vi "test server discover.vi"(8 "error in (no error)":errorcluster) -> (0 "error out":errorcluster, 3 "body":string)   [LabVIEW 2020, in "MCP Server tests.lvlib"]
doc: "server/discover (modern only) answers resultType complete, supportedVersions (all versions: 2026-07-28 and the legacy ones including 2025-11-25), the capabilities that initialize reports, _meta serverInfo and the caching hints. initialize stays legacy: asked for 2026-07-28 it answers the newest legacy version 2025-11-25, and 2025-11-25 is negotiable. The requests are sent with the LabVIEW HTTP Client directly."
uses:
  MCP Server tests.lvlib
  671d1c08-5dc6-4caa-967e-c1c9fcee9c7e.vi
  <vilib>/JDP Science/JSONtext/Next JSON Value.vi
  <vilib>/JDP Science/JSONtext/String Subset.vi
  <vilib>/JDP Science/JSONtext/Parsing/Advance past next JSON Value (inlined COPY).vi
  <vilib>/JDP Science/JSONtext/Parsing/Advance past whitespace.vi
  <vilib>/JDP Science/JSONtext/Parsing/Advance past String.vi
  <vilib>/JDP Science/JSONtext/Parsing/Advance past Number.vi
  <vilib>/JDP Science/JSONtext/Parsing/Advance past Line Ending.vi
  <vilib>/JDP Science/JSONtext/Parsing/Parse Full Path or Item Name.vi
  <vilib>/JDP Science/JSONtext/Parsing/Advance past Array.vi
  <vilib>/JDP Science/JSONtext/Parsing/Advance past Object.vi
  <vilib>/JDP Science/JSONtext/support/Error Cluster From Code.vi
  <vilib>/JDP Science/JSONtext/Offset/Find Item Locations by Path.vi
  <vilib>/JDP Science/JSONtext/JSON text to Variant.vi
  <vilib>/JDP Science/JSONtext/LVClass Serializer/JSONtext LVClass Serializer.lvclass
  <vilib>/addons/_JKI Toolkits/Caraya/classes/Test/Test.lvclass
  <vilib>/JDP Science/JSONtext/JSONtext.lvlib
  <vilib>/addons/_JKI Toolkits/Caraya/classes/Assert/Assert.lvclass
panel:
  out "lookup error":errorcluster
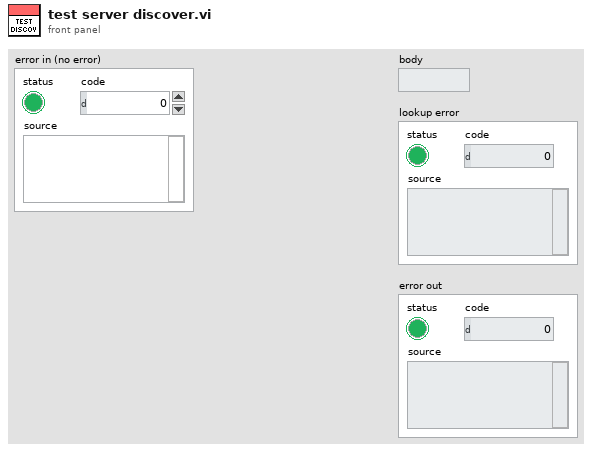
[diagram p1: front panel]
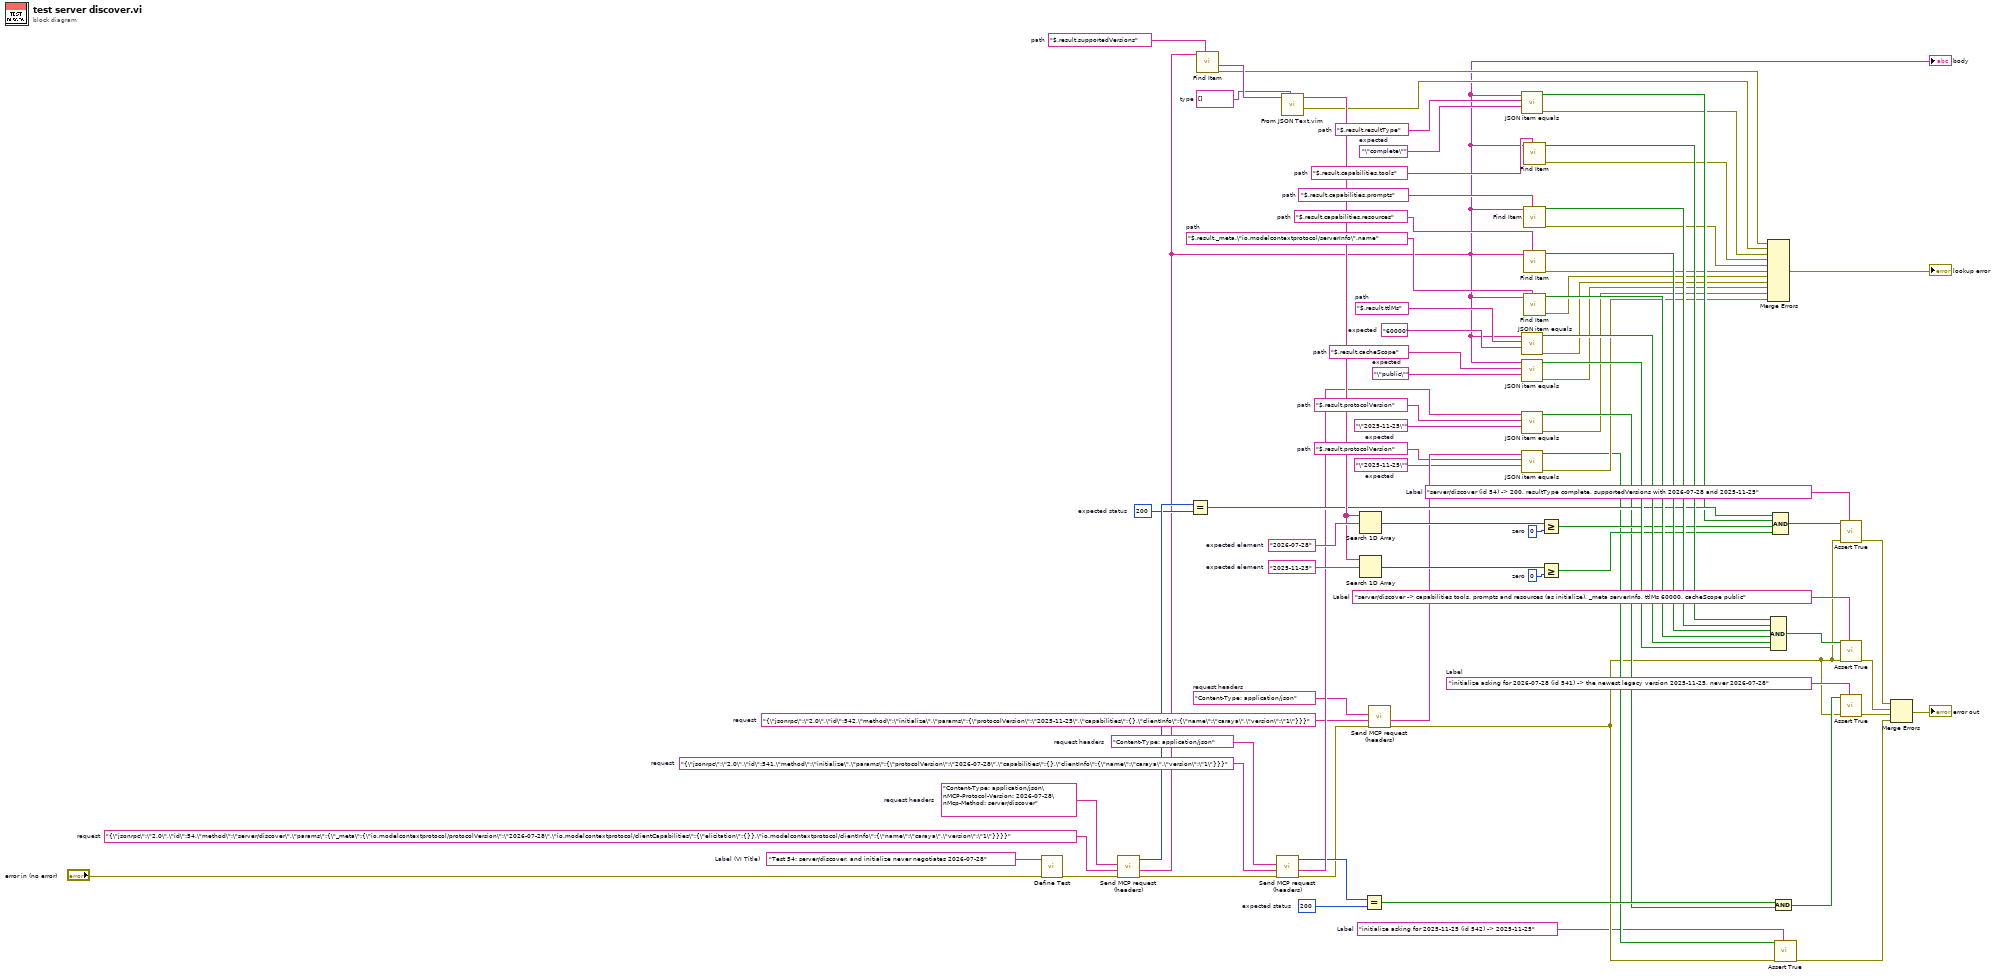
[diagram p0: block diagram]
diagram:
  w33 = "Content-Type: application/json"  # request headers
  w47 = "Content-Type: application/json"  # request headers
  w78 = "Content-Type: application/json\nMCP-Protocol-Version: 2026-07-28\nMcp-Method: server/discover"  # request headers
  w8 = "initialize asking for 2025-11-25 (id 542) -> 2025-11-25"  # Label
  w11 = "initialize asking for 2026-07-28 (id 541) -> the newest legacy version 2025-11-25, never 2026-07-28"  # Label
  w13 = "server/discover -> capabilities tools, prompts and resources (as initialize), _meta serverInfo, ttlMs 60000, cacheScope public"  # Label
  w15 = "server/discover (id 54) -> 200, resultType complete, supportedVersions with 2026-07-28 and 2025-11-25"  # Label
  w18 = "\"2025-11-25\""  # expected
  w19 = "$.result.protocolVersion"  # path
  w38 = "\"2025-11-25\""  # expected
  w39 = "$.result.protocolVersion"  # path
  w36 = 200  # expected status
  w63 = "\"public\""  # expected
  w64 = "$.result.cacheScope"  # path
  w65 = "60000"  # expected
  w66 = "$.result.ttlMs"  # path
  w71 = "$.result._meta.\"io.modelcontextprotocol/serverInfo\".name"  # path
  w72 = "$.result.capabilities.resources"  # path
  w73 = "$.result.capabilities.prompts"  # path
  w74 = "$.result.capabilities.tools"  # path
  w67 = "\"complete\""  # expected
  w68 = "$.result.resultType"  # path
  w61 = 200  # expected status
  w48 = 0  # zero
  w58 = "2025-11-25"  # expected element
  w50 = 0  # zero
  w60 = "2026-07-28"  # expected element
  w69 = string[] []  # type
  w75 = "$.result.supportedVersions"  # path
  w32 = "{\"jsonrpc\":\"2.0\",\"id\":542,\"method\":\"initialize\",\"params\":{\"protocolVersion\":\"2025-11-25\",\"capabilities\":{},\"clientInfo\":{\"name\":\"caraya\",\"version\":\"1\"}}}"  # request
  w46 = "{\"jsonrpc\":\"2.0\",\"id\":541,\"method\":\"initialize\",\"params\":{\"protocolVersion\":\"2026-07-28\",\"capabilities\":{},\"clientInfo\":{\"name\":\"caraya\",\"version\":\"1\"}}}"  # request
  w77 = "{\"jsonrpc\":\"2.0\",\"id\":54,\"method\":\"server/discover\",\"params\":{\"_meta\":{\"io.modelcontextprotocol/protocolVersion\":\"2026-07-28\",\"io.modelcontextprotocol/clientCapabilities\":{\"elicitation\":{}},\"io.modelcontextprotocol/clientInfo\":{\"name\":\"caraya\",\"version\":\"1\"}}}}"  # request
  w80 = "Test 54: server/discover, and initialize never negotiates 2026-07-28"  # Label (VI Title)
  n1 = call <vilib>:"Define Test.vi"("error in (no error)"="error in (no error)", "Label (VI Title)"=w80) -> ("error out"=w76:errorcluster)  [unwired: 8 in, 1 out]
  n2 = call "Send MCP request (headers).vi"("error in (no error)"=w76, "request"=w77, "request headers"=w78) -> ("error out"=w45:errorcluster, "response"=w3:string, "status code"=w62:i32)  [unwired: 5 in, 1 out]
  "body" <- w3
  n3 = Equal?(x=w62, y=w61) -> (x = y?=w44:bool)
  n4 = call <vilib>:"Find Item.vi"("$Path or Item Name"=w75, "JSON"=w3) -> ("error out"=w30:errorcluster, "<JSON>"=w70:string)  [unwired: 6 in, 2 out]
  n5 = call "Send MCP request (headers).vi"("error in (no error)"=w45, "request"=w46, "request headers"=w47) -> ("error out"=w31:errorcluster, "response"=w40:string, "status code"=w37:i32)  [unwired: 5 in, 1 out]
  n6 = call "From JSON Text.vim"("Data Type and Default Value"=w69, "JSON"=w70) -> ("error out"=w29:errorcluster, "Data out"=w59:string[])  [unwired: 8 in]
  n7 = Search 1D Array(1D array=w59, element=w60) -> (index of element=w51:i32)  [unwired: 1 in]
  n8 = Search 1D Array(1D array=w59, element=w58) -> (index of element=w49:i32)  [unwired: 1 in]
  n9 = Equal?(x=w37, y=w36) -> (x = y?=w35:bool)
  n10 = call "Send MCP request (headers).vi"("error in (no error)"=w31, "request"=w32, "request headers"=w33) -> ("error out"=w9:errorcluster, "response"=w20:string)  [unwired: 5 in, 2 out]
  n11 = call "JSON item equals.vi"("expected"=w67, "path"=w68, "JSON"=w3) -> ("error out"=w28:errorcluster, "equal?"=w43:bool)  [unwired: 6 in, 1 out]
  n12 = call "JSON item equals.vi"("expected"=w65, "path"=w66, "JSON"=w3) -> ("error out"=w23:errorcluster, "equal?"=w53:bool)  [unwired: 6 in, 1 out]
  n13 = call "JSON item equals.vi"("expected"=w63, "path"=w64, "JSON"=w3) -> ("error out"=w22:errorcluster, "equal?"=w52:bool)  [unwired: 6 in, 1 out]
  n14 = call "JSON item equals.vi"("expected"=w38, "path"=w39, "JSON"=w40) -> ("error out"=w21:errorcluster, "equal?"=w34:bool)  [unwired: 6 in, 1 out]
  n15 = call "JSON item equals.vi"("expected"=w18, "path"=w19, "JSON"=w20) -> ("error out"=w17:errorcluster, "equal?"=w10:bool)  [unwired: 6 in, 1 out]
  n16 = call <vilib>:"Find Item.vi"("$Path or Item Name"=w74, "JSON"=w3) -> ("error out"=w27:errorcluster, "Found"=w57:bool)  [unwired: 6 in, 2 out]
  n17 = call <vilib>:"Find Item.vi"("$Path or Item Name"=w73, "JSON"=w3) -> ("error out"=w26:errorcluster, "Found"=w56:bool)  [unwired: 6 in, 2 out]
  n18 = call <vilib>:"Find Item.vi"("$Path or Item Name"=w72, "JSON"=w3) -> ("error out"=w25:errorcluster, "Found"=w55:bool)  [unwired: 6 in, 2 out]
  n19 = call <vilib>:"Find Item.vi"("$Path or Item Name"=w71, "JSON"=w3) -> ("error out"=w24:errorcluster, "Found"=w54:bool)  [unwired: 6 in, 2 out]
  n20 = Greater Or Equal?(x=w51, y=w50) -> (x >= y?=w42:bool)
  n21 = Greater Or Equal?(x=w49, y=w48) -> (x >= y?=w41:bool)
  n22 = Merge Errors(w30, w29, w28, w27, w26, w25, w24, w23, w22, w21, w17) -> (→"lookup error":errorcluster)
  n23 = Compound Arithmetic op=AND(w57, w56, w55, w54, w53, w52) -> (w14:bool)
  n24 = Compound Arithmetic op=AND(w44, w43, w42, w41) -> (w16:bool)
  n25 = call <vilib>:"Assert True.vi"("Label"=w8, "error in (no error)"=w9, "True?"=w10) -> ("error out"=w4:errorcluster)  [unwired: 7 in, 1 out]
  n26 = Compound Arithmetic op=AND(w35, w34) -> (w12:bool)
  n27 = call <vilib>:"Assert True.vi"("Label"=w15, "error in (no error)"=w9, "True?"=w16) -> ("error out"=w7:errorcluster)  [unwired: 7 in, 1 out]
  n28 = call <vilib>:"Assert True.vi"("Label"=w13, "error in (no error)"=w9, "True?"=w14) -> ("error out"=w6:errorcluster)  [unwired: 7 in, 1 out]
  n29 = call <vilib>:"Assert True.vi"("Label"=w11, "error in (no error)"=w9, "True?"=w12) -> ("error out"=w5:errorcluster)  [unwired: 7 in, 1 out]
  n30 = Merge Errors(w7, w6, w5, w4) -> (→"error out":errorcluster)
